vi "Set_Command.vi"(8 "error in (no error)":errorcluster, 10 "Motor Control":dbl, 11 "Motor in":refnum<class "Motor.lvclass">) -> (0 "error out":errorcluster, 3 "Motor out":refnum<class "Motor.lvclass">)   [LabVIEW 2021, in "Motor.lvclass"]
uses:
  Motor.lvclass
  Motor.lvclass/Motor.ctl
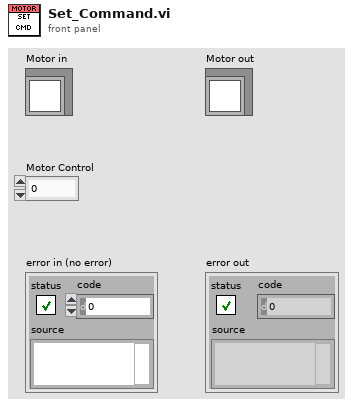
[diagram p1: front panel]
types:
  T1 = typedef "Motor.lvclass/Control_Mode.ctl" = enum16{"Speed", "Torque"}
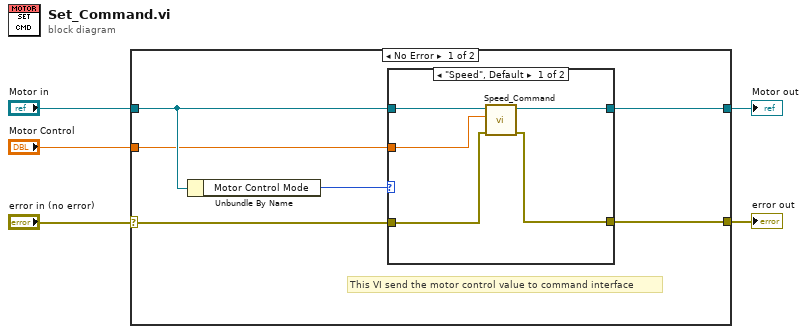
[diagram p0: block diagram]
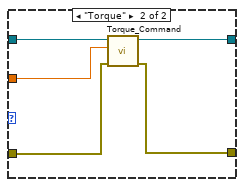
[diagram p2: hidden frame]
diagram:
  n1 = case shown="No Error" "error in (no error)" {
    selector: "error in (no error)" -> [w8 w23]
    tunnel: [w7 w23] -> w4
    tunnel: [w9 w22] -> w2
    tunnel: "Motor in" -> [w10 w22]
    tunnel: "Motor Control" -> [w6 _]
    frame No Error {
      # "This VI send the motor control value to command interface"
      n2 = Unbundle By Name(w10) -> ("Motor Control Mode"=w11:T1)
      n3 = case shown="\"Speed\", Default" w11 {
        tunnel: w10 -> [w16 w21]
        tunnel: [w15 w20] -> w9
        tunnel: w8 -> [w14 w19]
        tunnel: [w13 w18] -> w7
        tunnel: w6 -> [w12 w17]
        frame "Speed", Default {
          n4 = call "Speed_Command.vi"("error in (no error)"=w14, "Motor Control"=w12, "Motor in"=w16) -> ("error out"=w13:errorcluster, "Motor out"=w15:refnum<class "Motor.lvclass">)  [unwired: 7 in]
        }
        frame "Torque" {
          n5 = call "Torque_Command.vi"("error in (no error)"=w19, "Motor Control"=w17, "Motor in"=w21) -> ("error out"=w18:errorcluster, "Motor out"=w20:refnum<class "Motor.lvclass">)  [unwired: 7 in]
        }
      }
    }
    frame Error {
    }
  }
  "error out" <- w4
  "Motor out" <- w2
